vi "GetClientRect Wrapper Template.vi"(0 "hWnd":u64, 11 "error in":errorcluster) -> (4 "RECT":T1, 6 "return value":i32, 15 "error out":errorcluster)   [LabVIEW 2020]
doc: "Returns the client area of the window hWnd through user32.dll GetClientRect (stdcall, called in any thread): in CLIENT coordinates, so left and top are 0 and right and bottom are the width and height of the client area. The rectangle travels to the DLL as a RECT {LONG left, top, right, bottom}; right and bottom are exclusive. return value is the Win32 BOOL: non-zero on success. When error in carries an error the DLL is not called. Generated by scripts\\Build Win32 Wrappers.vi - do not edit by hand, rebuild it."
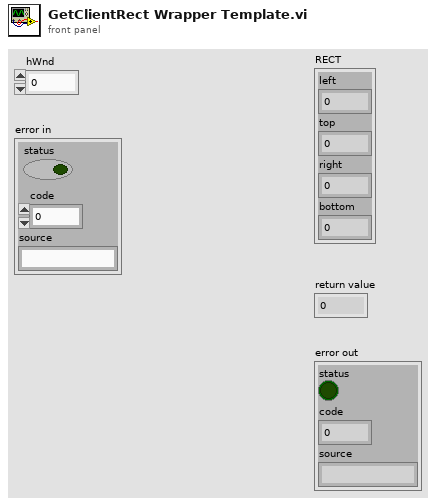
[diagram p1: front panel]
types:
  T1 = cluster{"left":i32, "top":i32, "right":i32, "bottom":i32}
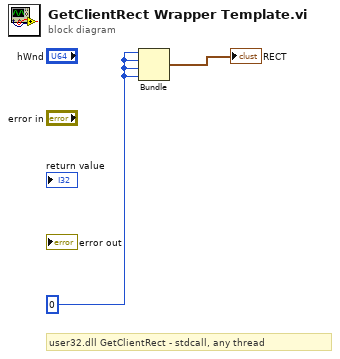
[diagram p0: block diagram]
diagram:
  w2 = 0
  # "user32.dll GetClientRect - stdcall, any thread"
  n1 = Bundle(w2, w2, w2, w2) -> (→"RECT":cluster{i32, i32, i32, i32})  [unwired: 1 in]
